vi "Read CSM API with lvcsm Support.vi"(6 "Config Path (\"\" For Lvcsm File)":path, 7 "Current Module (\"\" to Generate an ID)":string, 8 "error in (no error)":errorcluster, 9 "Force? (F)":bool, 11 "CSM Name":string) -> (0 "error out":errorcluster, 3 "CSMAPI List":string[](array[string]))   [LabVIEW 2017, in "CSM-Helper API with lvcsm Support.lvlib"]
uses:
  CSM-Helper API with lvcsm Support.lvlib
  CSM-Helper.lvclass
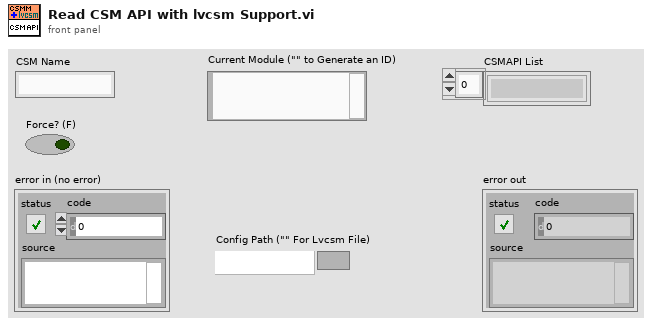
[diagram p1: front panel]
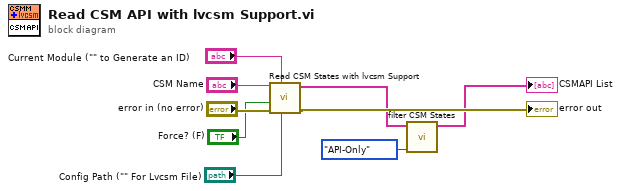
[diagram p0: block diagram]
diagram:
  n1 = call "Read CSM States with lvcsm Support.vi"("Config Path (\"\" For Lvcsm File)"="Config Path (\"\" For Lvcsm File)", "Current Module (\"\" to Generate an ID)"="Current Module (\"\" to Generate an ID)", "error in (no error)"="error in (no error)", "Force? (F)"="Force? (F)", "CSM Name"="CSM Name") -> ("error out"=→"error out":errorcluster, "CSMAPI List"=w2:string[])  [unwired: 5 in]
  n2 = call "filter CSM States.vi"("Interface-Filter"=enum16{"API-Only", "UserDef States", "All"}."API-Only", "Array"=w2) -> ("filtered array"=→"CSMAPI List":string[])  [unwired: 9 in]
